vi "set Swept SA - Sweep Count.vi"(8 "error in (no error)":errorcluster, 10 "Sweep Count":u32, 11 "Interface_Spectrum in":refnum<class "Interface_Spectrum.lvclass">) -> (0 "error out":errorcluster, 3 "Interface_Spectrum out":refnum<class "Interface_Spectrum.lvclass">)   [LabVIEW 2023, in "Spectrum Analyzer.lvlib" / "Interface_Spectrum.lvclass"]
doc: "This command defines the number of sweeps started with single sweep, which are\nused for calculating the average or maximum value. If the values 0 or 1 are set, one\nsweep is performed.\n\n* For FSV-40\n1) Parameters:\n<NumberSweeps> 0 to 32767\n *RST: 0 (GSM: 200, PHN:1)\nExample: SWE:COUN 64\n Sets the number of sweeps to 64.\n INIT:CONT OFF\n Switches to single sweep mode.\n INIT;*WAI\n Starts a sweep and waits for its end."
uses:
  Interface_Spectrum.lvclass
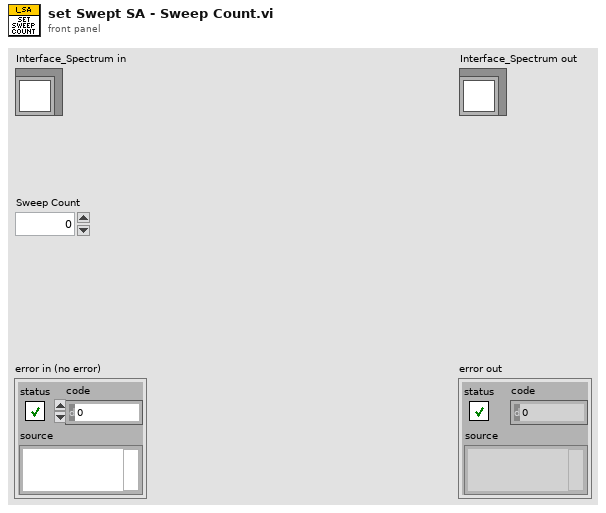
[diagram p1: front panel]
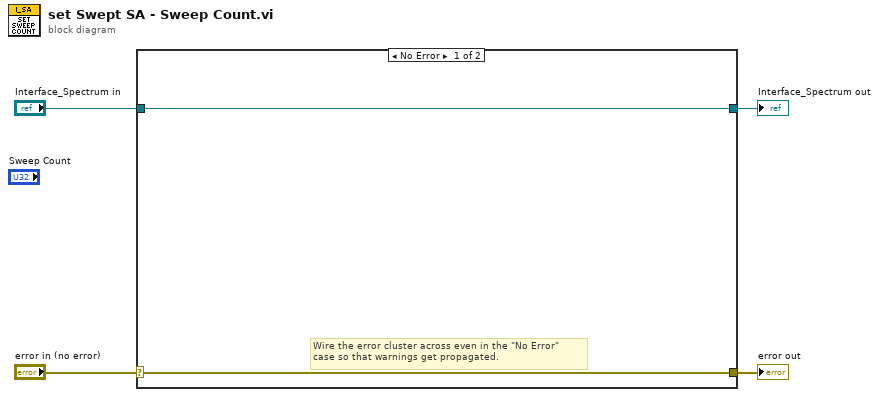
[diagram p0: block diagram]
diagram:
  n1 = case shown="No Error" "error in (no error)" {
    selector: "error in (no error)" -> [w5 w8]
    tunnel: [w5 w8] -> w3
    tunnel: [w6 w7] -> w1
    tunnel: "Interface_Spectrum in" -> [w6 w7]
    frame No Error {
      # "Wire the error cluster across even in the \"No Error\"\ncase so that warnings get propagated."
    }
    frame Error {
    }
  }
  "error out" <- w3
  "Interface_Spectrum out" <- w1
